vi "Get Recursive Owned VIs List.vi"(0 "Parent[]":refnum<vi>[](array[refnum]), 11 "error in":errorcluster) -> (4 "Children[]":refnum<vi>[](array[refnum]), 15 "error out":errorcluster)   [LabVIEW 2022 SP3, in "Springboard TLB`.lvlib"]
uses:
  Springboard TLB`.lvlib
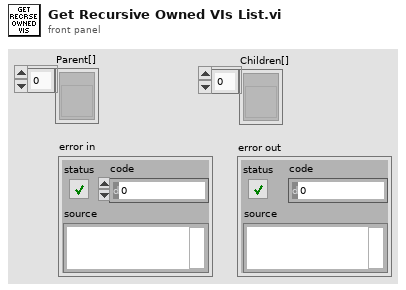
[diagram p1: front panel]
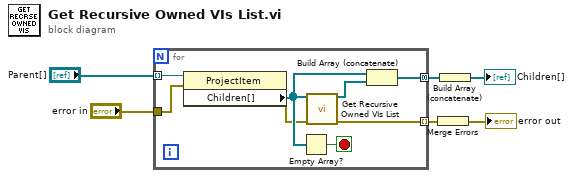
[diagram p0: block diagram]
diagram:
  n1 = for {
    tunnel: "Parent[]" -> [w14] mode=indexing
    tunnel: [w11] -> w6 mode=concatenating
    tunnel: "error in" -> [w9]
    tunnel: [w7] -> w2 mode=indexing
    stop <- w13 stop-if-true
    n2 = property class="ProjectItem"(reference=w14, error in=w9) -> (error out=w8:errorcluster, "Children[]"=w12:refnum<vi>[])  [unwired: 1 out]
    n3 = Empty Array?(array=w12) -> (empty?=w13:bool)
    n4 = call "Get Recursive Owned VIs List.vi"("Parent[]"=w12, "error in"=w8) -> ("Children[]"=w10:refnum<vi>[], "error out"=w7:errorcluster)  [unwired: 12 in]
    n5 = Build Array (concatenate)(w12, w10) -> (w11:refnum<vi>[])
  }
  n6 = Merge Errors(w2) -> (→"error out":errorcluster)
  n7 = Build Array (concatenate)(w6) -> (→"Children[]":refnum<vi>[])
